vi "Create Source.vi"(7 "VolatusAPI":refnum<class "VolatusAPI.lvclass">, 8 "error in (no error)":errorcluster, 10 "Type":string, 11 "Config":refnum<class "Config Element.lvclass">) -> (0 "error out":errorcluster, 3 "EStop Source":refnum<class "EStop Source.lvclass">)   [LabVIEW 2025, in "VolatusControl.lvlib" / "EStop Module.lvclass"]
uses:
  EStop Module.lvclass
  EStop Module.lvclass/EStop Module.ctl
  EStop Source/EStop Source.lvclass
  lv-cdm/CDM-Config/Config Element/Config Element.lvclass
  Volatus/VolatusAPI/VolatusAPI.lvclass
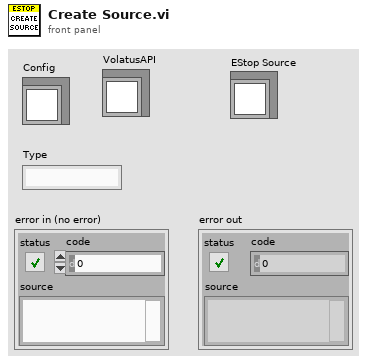
[diagram p1: front panel]
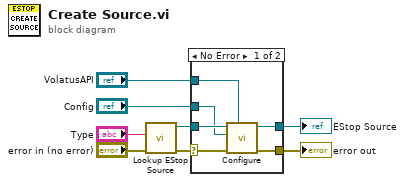
[diagram p0: block diagram]
diagram:
  n1 = call "Lookup EStop Source.vi"("error in (no error)"="error in (no error)", "Source Type"="Type") -> ("error out"=w4:errorcluster, "Source"=w7:refnum<class "EStop Source.lvclass">)  [unwired: 8 in]
  n2 = case shown="No Error" w4 {
    selector: w4 -> [w11 w15]
    tunnel: w7 -> [w14 _]
    tunnel: "Config" -> [w13 _]
    tunnel: "VolatusAPI" -> [w12 _]
    tunnel: [w10 w15] -> w1
    tunnel: [w9 _] -> w3
    frame No Error {
      n3 = call-dynamic "Configure.vi"("VolatusAPI"=w12, "error in (no error)"=w11, "Config Element"=w13, "EStop Source in"=w14) -> ("error out"=w10:errorcluster, "EStop Source out"=w9:refnum<class "EStop Source.lvclass">)  [unwired: 6 in]
    }
    frame Error {
    }
  }
  "error out" <- w1
  "EStop Source" <- w3
